vi "test resource custom uri.vi"(8 "error in (no error)":errorcluster) -> (0 "error out":errorcluster, 3 "body":string)   [LabVIEW 2020, in "MCP Server tests.lvlib"]
doc: "A resource added with the uri input of Add Resource (File).vi is listed and read under exactly that uri. Add Fixture Custom URI.vi registers fixture_utf8.txt as test://fixture-text. resources/list (id 741) lists test://fixture-text; resources/read of test://fixture-text (id 742) returns contents[0] with that uri, mimeType text/plain and the same text as the read of the derived uri labview://fixture_utf8 (id 743); a modern resources/read of it with Mcp-Name test://fixture-text (id 744) is answered HTTP 200, resultType complete. The requests are sent with the LabVIEW HTTP Client directly."
uses:
  MCP Server tests.lvlib
  <vilib>/addons/_JKI Toolkits/Caraya/classes/Test/Test.lvclass
  <vilib>/addons/_JKI Toolkits/Caraya/classes/Assert/Assert.lvclass
panel:
  out "lookup error":errorcluster
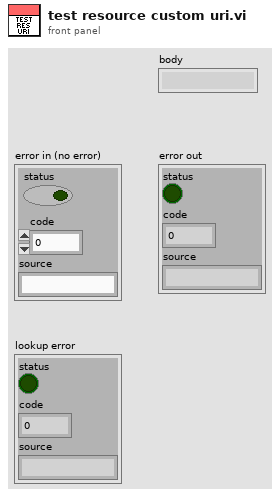
[diagram p1: front panel]
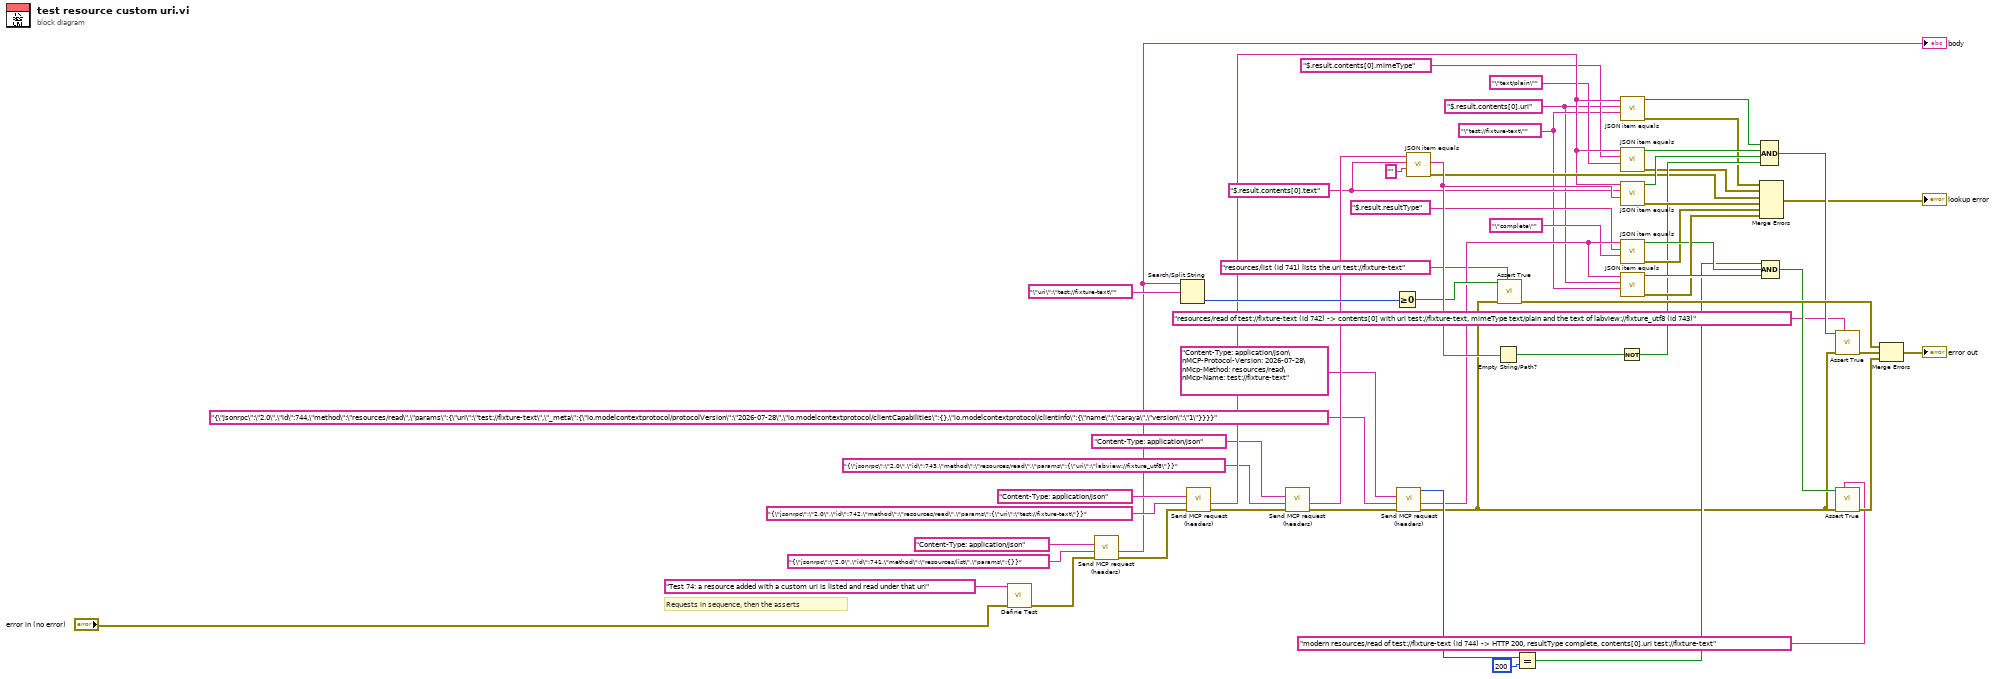
[diagram p0: block diagram]
diagram:
  w19 = "$.result.contents[0].text" ("path")
  w16 = "\"test://fixture-text\"" ("expected")
  w15 = "$.result.contents[0].uri" ("path")
  # "Requests in sequence, then the asserts"
  n1 = call <vilib>:"Define Test.vi"("error in (no error)"="error in (no error)", "Label (VI Title)"="Test 74: a resource added with a custom uri is listed and read under that uri") -> ("error out"=w27:errorcluster)  [unwired: 8 in, 1 out]
  n2 = call "Send MCP request (headers).vi"("error in (no error)"=w27, "request"="{\"jsonrpc\":\"2.0\",\"id\":741,\"method\":\"resources/list\",\"params\":{}}", "request headers"="Content-Type: application/json") -> ("error out"=w28:errorcluster, "response"=w2:string)  [unwired: 5 in, 2 out]
  "body" <- w2
  n3 = Search/Split String(string=w2, search string/char (-)="\"uri\":\"test://fixture-text\"" ("listed uri")) -> (offset of match=w36:i32)  [unwired: 1 in, 2 out]
  n4 = call "Send MCP request (headers).vi"("error in (no error)"=w28, "request"="{\"jsonrpc\":\"2.0\",\"id\":742,\"method\":\"resources/read\",\"params\":{\"uri\":\"test://fixture-text\"}}", "request headers"="Content-Type: application/json") -> ("error out"=w29:errorcluster, "response"=w30:string)  [unwired: 5 in, 2 out]
  n5 = call "Send MCP request (headers).vi"("error in (no error)"=w29, "request"="{\"jsonrpc\":\"2.0\",\"id\":743,\"method\":\"resources/read\",\"params\":{\"uri\":\"labview://fixture_utf8\"}}", "request headers"="Content-Type: application/json") -> ("error out"=w31:errorcluster, "response"=w32:string)  [unwired: 5 in, 2 out]
  n6 = Greater Or Equal To 0?(x=w36) -> (x >= 0?=w37:bool)
  n7 = call "Send MCP request (headers).vi"("error in (no error)"=w31, "request"="{\"jsonrpc\":\"2.0\",\"id\":744,\"method\":\"resources/read\",\"params\":{\"uri\":\"test://fixture-text\",\"_meta\":{\"io.modelcontextprotocol/protocolVersion\":\"2026-07-28\",\"io.modelcontextprotocol/clientCapabilities\":{},\"io.modelcontextprotocol/clientInfo\":{\"name\":\"caraya\",\"version\":\"1\"}}}}", "request headers"="Content-Type: application/json\nMCP-Protocol-Version: 2026-07-28\nMcp-Method: resources/read\nMcp-Name: test://fixture-text") -> ("error out"=w33:errorcluster, "response"=w34:string, "status code"=w35:i32)  [unwired: 5 in, 1 out]
  n8 = call "JSON item equals.vi"("expected"="", "path"=w19, "JSON"=w32) -> ("error out"=w42:errorcluster, "item"=w43:string)  [unwired: 6 in, 1 out]
  n9 = Empty String/Path?(string/path=w43) -> (empty?=w44:bool)
  n10 = call <vilib>:"Assert True.vi"("Label"="resources/list (id 741) lists the uri test://fixture-text", "error in (no error)"=w33, "True?"=w37) -> ("error out"=w55:errorcluster)  [unwired: 7 in, 1 out]
  n11 = Equal?(x=w35, y=200 ("expected status")) -> (x = y?=w48:bool)
  n12 = Not(x=w44) -> (.not. x?=w45:bool)
  n13 = call "JSON item equals.vi"("expected"=w16, "path"=w15, "JSON"=w30) -> ("error out"=w38:errorcluster, "equal?"=w39:bool)  [unwired: 6 in, 1 out]
  n14 = call "JSON item equals.vi"("expected"="\"text/plain\"", "path"="$.result.contents[0].mimeType", "JSON"=w30) -> ("error out"=w40:errorcluster, "equal?"=w41:bool)  [unwired: 6 in, 1 out]
  n15 = call "JSON item equals.vi"("expected"=w43, "path"=w19, "JSON"=w30) -> ("error out"=w46:errorcluster, "equal?"=w47:bool)  [unwired: 6 in, 1 out]
  n16 = call "JSON item equals.vi"("expected"="\"complete\"", "path"="$.result.resultType", "JSON"=w34) -> ("error out"=w49:errorcluster, "equal?"=w50:bool)  [unwired: 6 in, 1 out]
  n17 = call "JSON item equals.vi"("expected"=w16, "path"=w15, "JSON"=w34) -> ("error out"=w51:errorcluster, "equal?"=w52:bool)  [unwired: 6 in, 1 out]
  n18 = Merge Errors(w38, w40, w42, w46, w49, w51) -> (→"lookup error":errorcluster)
  n19 = Compound Arithmetic op=AND(w39, w41, w47, w45) -> (w53:bool)
  n20 = Compound Arithmetic op=AND(w48, w50, w52) -> (w54:bool)
  n21 = call <vilib>:"Assert True.vi"("Label"="resources/read of test://fixture-text (id 742) -> contents[0] with uri test://fixture-text, mimeType text/plain and the text of labview://fixture_utf8 (id 743)", "error in (no error)"=w33, "True?"=w53) -> ("error out"=w56:errorcluster)  [unwired: 7 in, 1 out]
  n22 = call <vilib>:"Assert True.vi"("Label"="modern resources/read of test://fixture-text (id 744) -> HTTP 200, resultType complete, contents[0].uri test://fixture-text", "error in (no error)"=w33, "True?"=w54) -> ("error out"=w57:errorcluster)  [unwired: 7 in, 1 out]
  n23 = Merge Errors(w55, w56, w57) -> (→"error out":errorcluster)
